vi "Untitled 1.vi"() -> ()   [LabVIEW 2026]
panel:
  in  "Numeric 2":dbl
  out "Numeric":dbl
  in  "Boolean":bool
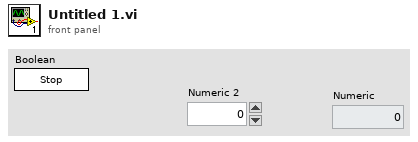
[diagram p1: front panel]
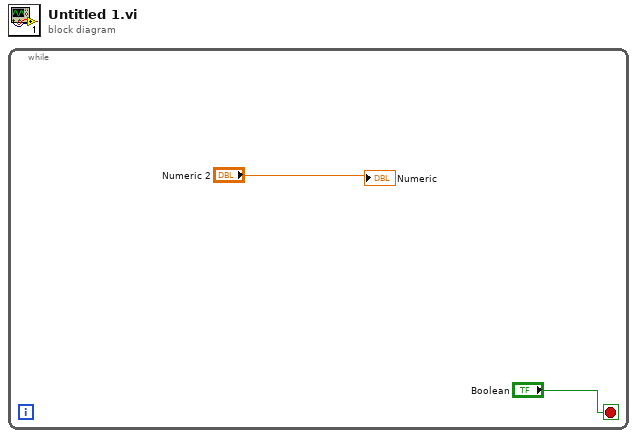
[diagram p0: block diagram]
diagram:
  n1 = while {
    stop <- "Boolean" stop-if-true
    "Numeric" <- "Numeric 2"
  }
